vi "Initialize.vi"(8 "error in":errorcluster, 11 "Plugin in":refnum<class "Nominal-TDMS-Upload.lvclass">) -> (0 "error out":errorcluster, 3 "Plugin out":refnum<class "Nominal-TDMS-Upload.lvclass">)   [LabVIEW 2026, in "Nominal-TDMS-Upload.lvlib" / "Nominal-TDMS-Upload.lvclass"]
uses:
  Nominal-TDMS-Upload.lvclass
  <vilib>/FlexLogger/SDK/PluginSDK.lvlibp/PEFClasses/SDK/Processing Element/Timing Parameters.ctl
  <vilib>/FlexLogger/SDK/PluginSDK.lvlibp/PEFClasses/SDK/Processing Element/Timing Method.ctl
  <vilib>/FlexLogger/SDK/PluginSDK.lvlibp/PEFClasses/SDK/Plugin/ParameterAccess/Write String.vi
  <vilib>/FlexLogger/SDK/PluginSDK.lvlibp/PEFClasses/SDK/Plugin/Plugin.lvclass
  <vilib>/FlexLogger/SDK/PluginSDK.lvlibp/PEFClasses/SDK/Processing Element/Processing Element.lvclass
  <vilib>/FlexLogger/SDK/PluginSDK.lvlibp/PEFClasses/SDK/Plugin/ParameterAccess/Write Command.vi
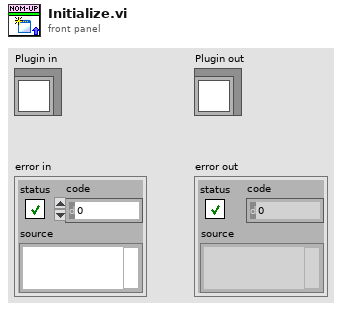
[diagram p1: front panel]
types:
  T1 = typedef "PluginSDK.lvlibp/Processing Element.lvclass/Timing Parameters.ctl" = cluster{"Timing Method":T2, "Timing Period (ms)":i32}
  T2 = typedef "PluginSDK.lvlibp/Processing Element.lvclass/Timing Method.ctl" = enum16{"Periodic", "Immediate", "On Data Ready", "Triggered"}
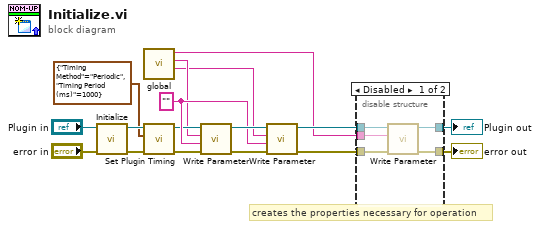
[diagram p0: block diagram]
diagram:
  w11 = "" ("Value")
  # "creates the properties necessary for operation"
  n1 = call-parent "Initialize.vi"("error in (no error)"="error in", "Plugin in"="Plugin in") -> ("error out"=w14:errorcluster, "Plugin out"=w15:refnum<class "Nominal-TDMS-Upload.lvclass">)  [unwired: 8 in]
  n2 = call "global.vi"() -> ("dataset RID"=w6:string, "API Key"=w7:string, "command"=w1:string)  [unwired: 9 in]
  n3 = call <vilib>:"Set Plugin Timing.vi"("error in (no error)"=w14, "Timing Parameters"=T1 {"Timing Method"=enum."Periodic", "Timing Period (ms)"=1000}, "Plugin in"=w15) -> ("error out"=w10:errorcluster, "Plugin out"=w9:refnum<class "Nominal-TDMS-Upload.lvclass">)  [unwired: 7 in]
  n4 = call-poly <vilib>:"Write Parameter.vi"("error in (no error)"=w10, "Value"=w11, "Name"=w7, "Plugin in"=w9) -> ("error out"=w13:errorcluster, "Plugin out"=w12:refnum<class "Nominal-TDMS-Upload.lvclass">)  [unwired: 6 in]
  n5 = call-poly <vilib>:"Write Parameter.vi"("error in (no error)"=w13, "Value"=w11, "Name"=w6, "Plugin in"=w12) -> ("error out"=w8:errorcluster, "Plugin out"=w3:refnum<class "Nominal-TDMS-Upload.lvclass">)  [unwired: 6 in]
  n6 = disable-structure shown="Disabled" {
    disable-tunnel: w8 -> [w22 w24]
    disable-tunnel: [w21 w24] -> w4
    disable-tunnel: w3 -> [w20 w23]
    disable-tunnel: [w19 w23] -> w2
    disable-tunnel: w1 -> [w18 _]
    frame Disabled {
      n7 = call-poly <vilib>:"Write Parameter.vi"("error in (no error)"=w22, "Name"=w18, "Plugin in"=w20) -> ("error out"=w21:errorcluster, "Plugin out"=w19:refnum<class "Nominal-TDMS-Upload.lvclass">)  [unwired: 7 in]
    }
    frame Enabled {
    }
  }
  "error out" <- w4
  "Plugin out" <- w2
